vi "CO change Ant Pol.vi"(8 "error in (no error)":errorcluster caption="에러 입력(에러 없음)", 10 "Antenna Pol":enum16{"H", "V"}(ring), 11 "Instrument Manager 입력":refnum<class "Instrument Manager.lvclass">) -> (0 "error out":errorcluster caption="에러 출력", 3 "Instrument Manager 출력":refnum<class "Instrument Manager.lvclass">)   [LabVIEW 2023, in "Instrument Manager.lvclass"]
uses:
  Instrument Manager.lvclass
  Module/Turn Table and Mast Control/Class/CO3000/CO3000.lvclass
  C:/Users/HCT-3320/Documents/Instrument Manger/Module/Turn Table and Mast Control/Interface Class/Mast/Interface - Mast.lvclass
  Module/Turn Table and Mast Control/Interface Class/Mast/Interface - Mast.lvclass
  Instrument Manager.lvclass/Instrument Manager.ctl
  Module/Turn Table and Mast Control/Class/CO3000/CO3000.lvclass/CO3000.ctl
  d552f2b8-8be9-4d15-8ce9-d93ff2c16b38.vi
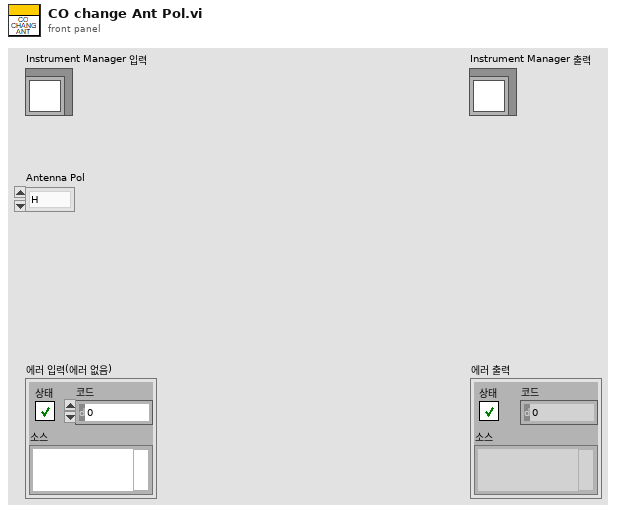
[diagram p1: front panel]
types:
  T1 = cluster{"Anritsu Call Box":refnum<class "Anritsu Call Box.lvclass">, "Spectrum Analyzer":refnum<class "Interface_Spectrum.lvclass">, "RF Switch Box":refnum<class "RF Filter Box.lvclass">, "Turn Table":refnum<class "Interface - Turn Table.lvclass">, "Mast":refnum<class "Interface - Mast.lvclass">, "3D Controller":refnum<class "Interface_3D Controller.lvclass">}
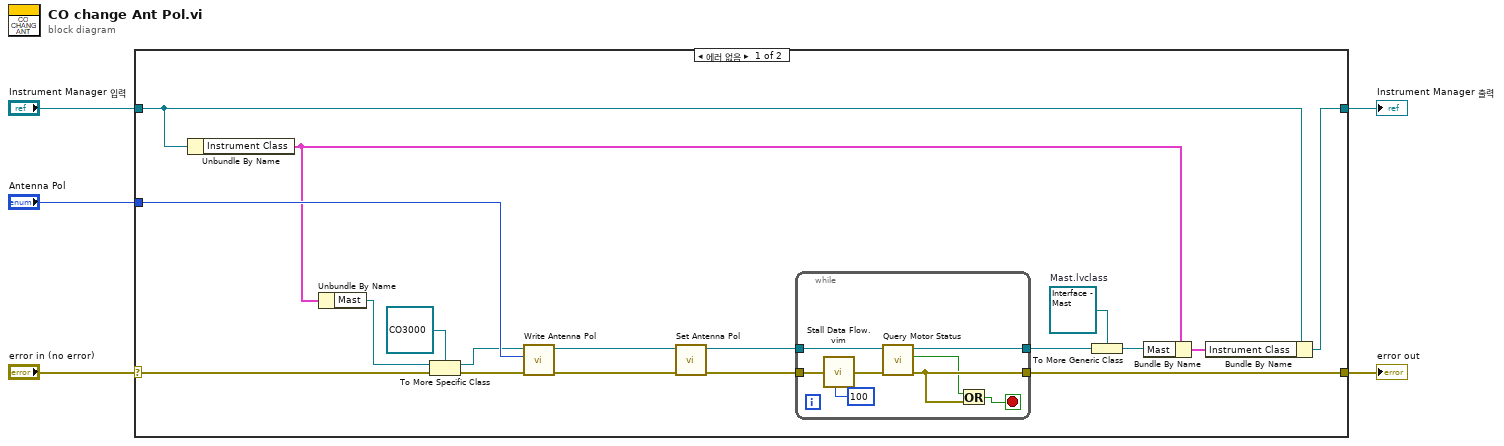
[diagram p0: block diagram]
diagram:
  n1 = case shown="에러 없음" "error in (no error)" {
    selector: "error in (no error)" -> [w20 w33]
    tunnel: [w6 w33] -> w4
    tunnel: [w23 w32] -> w2
    tunnel: "Instrument Manager 입력" -> [w22 w32]
    tunnel: "Antenna Pol" -> [w18 _]
    frame No Error {
      w10 = refnum<class "Interface - Mast.lvclass"> refnum  # Mast.lvclass
      n2 = Unbundle By Name(w22) -> ("Instrument Class"=w9:T1)
      n3 = Unbundle By Name(w9) -> ("Mast"=w21:refnum<class "Interface - Mast.lvclass">)
      n4 = To More Specific Class(target class=refnum<class "CO3000.lvclass"> refnum ("CO3000 in"), reference=w21, error in=w20) -> (specific class reference=w16:refnum<class "CO3000.lvclass">, error out=w17:errorcluster)
      n5 = call "Write Antenna Pol.vi"("error in (no error)"=w17, "Antenna Pol"=w18, "CO3000 in"=w16) -> ("error out"=w14:errorcluster, "CO3000 out"=w15:refnum<class "CO3000.lvclass">)  [unwired: 7 in]
      n6 = call-dynamic "Set Antenna Pol.vi"("error in (no error)"=w14, "CO3000 in"=w15) -> ("error out"=w12:errorcluster, "CO3000 out"=w13:refnum<class "CO3000.lvclass">)  [unwired: 8 in]
      n7 = while {
        tunnel: w13 -> [w31]
        tunnel: w12 -> [w30]
        tunnel: [w26] -> w6
        tunnel: [w27] -> w7
        stop <- w24 stop-if-true
        n8 = call "Stall Data Flow.vim"("value in"=w30, "milliseconds to wait"=u32 100) -> ("value out"=w28:errorcluster)  [unwired: 1 out]
        n9 = call-dynamic "Query Motor Status.vi"("error in (no error)"=w28, "CO3000 in"=w31) -> ("error out"=w26:errorcluster, "Motor Stop?"=w25:bool, "CO3000 out"=w27:refnum<class "CO3000.lvclass">)  [unwired: 7 in]
        n10 = Or(x=w25, y=w26) -> (x .or. y?=w24:bool)
      }
      n11 = To More Generic Class(target class=w10, reference=w7) -> (generic class reference=w11:refnum<class "Interface - Mast.lvclass">)
      n12 = Bundle By Name(cluster=w9, "Mast"=w11) -> (w8:T1)
      n13 = Bundle By Name(cluster=w22, "Instrument Class"=w8) -> (w23:refnum<class "Instrument Manager.lvclass">)
    }
    frame Error {
    }
  }
  "error out" <- w4
  "Instrument Manager 출력" <- w2
